vi "Populate Tree with Delimited Strings_csm.vi"(5 "Use Child Only?":bool, 7 "Default Symbol":i32=37, 8 "error in (no error)":errorcluster, 9 "Delimiter":string=".", 10 "Items (Delimited)":string[][](array[string]), 11 "Tree Control":refnum<vi>) -> (0 "error out":errorcluster, 2 "Parents Added":string[](array[string]), 3 "Tree Control Dup":refnum<vi>)   [LabVIEW 2017, in "csm-ui-support.lvlib"]
uses:
  csm-ui-support.lvlib
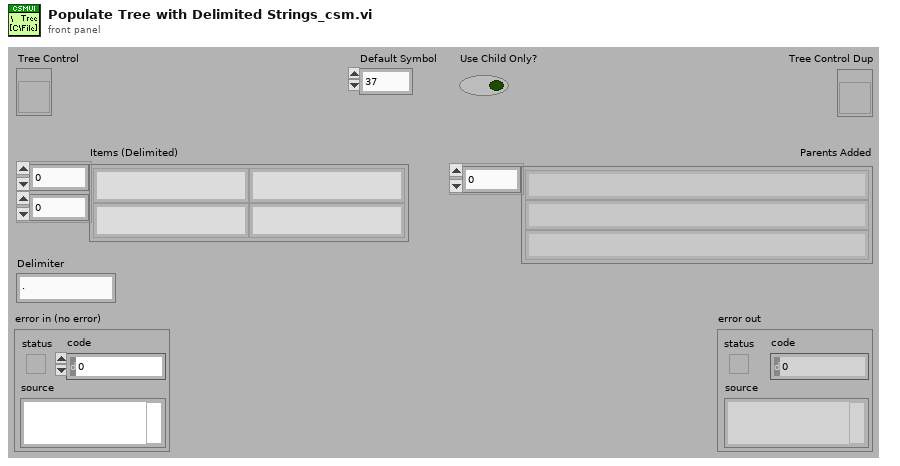
[diagram p1: front panel]
types:
  T1 = cluster{"Left Cell String":string, "Child Text":string[], "Child Tag":string, "Item Indent":i32, "Child Only?":bool, "Glyph Index":i32}[]
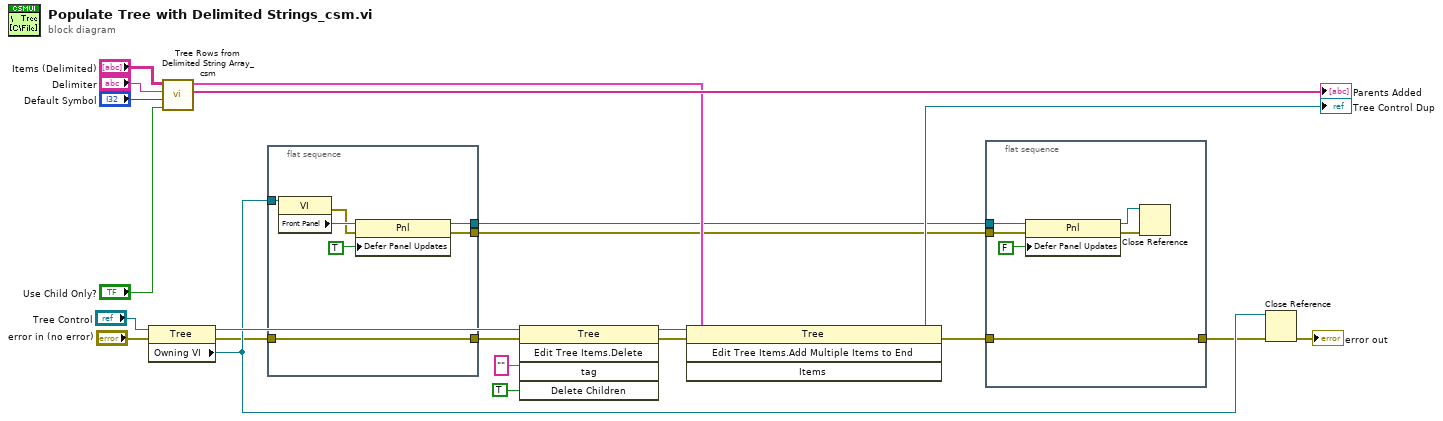
[diagram p0: block diagram]
diagram:
  n1 = property class="Tree"(reference="Tree Control", error in="error in (no error)") -> (reference out=w9:refnum<vi>, error out=w3:errorcluster, "Owning VI"=w7:refnum<vi>)
  n2 = call "Tree Rows from Delimited String Array_csm.vi"("Use Child Only? (F)"="Use Child Only?", "Default Symbol"="Default Symbol", "Delimiter"="Delimiter", "Items (Delimited)"="Items (Delimited)") -> ("Parent Tag Added[]"=→"Parents Added":string[], "Item to Add[]"=w11:T1)  [unwired: 6 in]
  n3 = flat-sequence {
    tunnel: w7 -> [w29]
    tunnel: [w25] -> w6
    tunnel: [w24] -> w5
    tunnel: [w23] -> w4
    tunnel: w3 -> [w23]
    frame #0 {
      n4 = property class="VI"(reference=w29) -> (error out=w26:errorcluster, "Front Panel"=w28:refnum<vi>)  [unwired: 1 in, 1 out]
      n5 = property class="Pnl"(reference=w28, error in=w26, "Defer Panel Updates"=TRUE) -> (reference out=w24:refnum<vi>, error out=w25:errorcluster)
    }
  }
  n6 = invoke on="Invoke Node" class="Tree" method="Edit Tree Items.Delete"(reference=w9, error in=w4, "tag"="" ("Tag"), "Delete Children"=TRUE ("Delete Children?")) -> (reference out=w13:refnum<vi>, error out=w12:errorcluster)  [unwired: 1 in, 3 out]
  n7 = invoke on="Invoke Node" class="Tree" method="Edit Tree Items.Add Multiple Items to End"(reference=w13, error in=w12, "Items"=w11) -> (reference out=→"Tree Control Dup":refnum<vi>, error out=w1:errorcluster)  [unwired: 1 in, 2 out]
  n8 = flat-sequence {
    tunnel: w6 -> [w34]
    tunnel: w5 -> [w33]
    tunnel: [w30] -> w2
    tunnel: w1 -> [w30]
    frame #0 {
      n9 = property class="Pnl"(reference=w33, error in=w34, "Defer Panel Updates"=FALSE) -> (reference out=w31:refnum<vi>, error out=w32:errorcluster)
      n10 = Close Reference(reference=w31, error in (no error)=w32) -> ()  [unwired: 1 out]
    }
  }
  n11 = Close Reference(reference=w7, error in (no error)=w2) -> (error out=→"error out":errorcluster)
